vi "Test_HelloWorld_InvalidUtf8Encoding.vi"() -> (0 "Array of Error Description":T1)   [LabVIEW 2019]
uses:
  gRPC_ATS/TestUtility/utility.llb/array of error description.ctl
  gRPC_ATS/TestUtility/utility.llb/error description.ctl
  gRPC_ATS/TestUtility/utility.llb/error type.ctl
  examples/helloworld/helloworld_client/RPC Messages/helloworld_HelloRequest.ctl
  690210b7-9fc1-4805-899f-f09b8e1640af.vi
  86c0777a-bec3-4a03-9553-2f9525a5fa02.vi
  <vilib>/gRPC/LabVIEW gRPC Library/Server API/Translate Protobuf Error.vi
  <vilib>/AdvancedString/1D String Array to Delimited String.vi
  <vilib>/gRPC/LabVIEW gRPC Library/Server API/Server/Get Server DLL Path.vi
  examples/helloworld/helloworld_client/helloworld_client.lvlib
panel:
  out "Pass":bool
  in  "error in (no error)":errorcluster
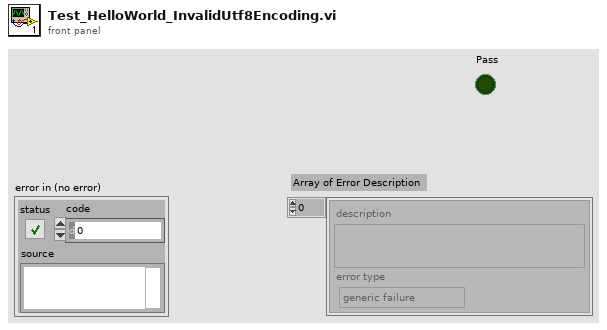
[diagram p1: front panel]
types:
  T1 = typedef "array of error description.ctl" = T2[]
  T2 = typedef "error description.ctl" = cluster{"description":string, "error type":T3}
  T3 = typedef "error type.ctl" = enum32{"generic failure", "boundary case", "precision", "expected error"}
  T4 = typedef "helloworld_client.lvlib/helloworld_HelloRequest.ctl" = cluster{"name":string}
  T5 = typedef "grpc-lvsupport-release.lvlib/grpcId.ctl" = u64
  T6 = typedef "grpc-lvsupport-release.lvlib/Any.ctl" = cluster{"Type Url":string, "Bytes":u8[]}
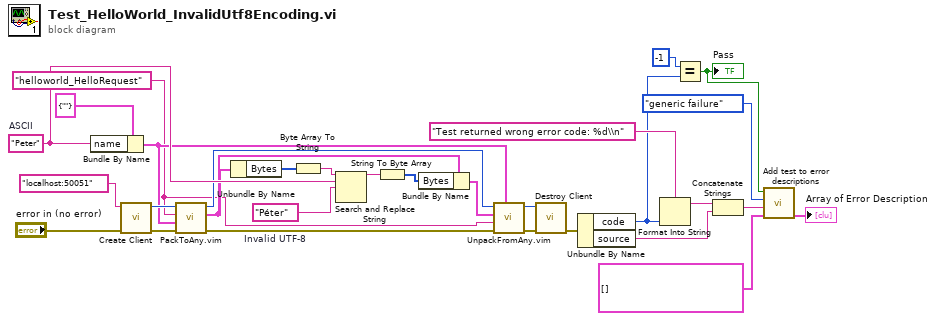
[diagram p0: block diagram]
diagram:
  w16 = "Péter"  # Invalid UTF-8
  w17 = "Peter"  # ASCII
  w9 = "helloworld_HelloRequest" ("Message Type")
  n1 = Bundle By Name(cluster=T4 {"name"=""} ("helloworld_HelloRequest"), "name"=w17) -> (w11:T4)
  n2 = call "Create Client.vi"("error in"="error in (no error)", "address"="localhost:50051") -> ("error out"=w23:errorcluster, "gRPC ID Out"=w22:T5)  [unwired: 8 in]
  n3 = call "PackToAny.vim"("error in"=w23, "Data To Pack"=w11, "Message Type"=w9, "gRPCid in"=w22) -> ("error out"=w7:errorcluster, "Any"=w14:T6, "gRPCid out"=w10:u64)  [unwired: 5 in]
  n4 = Unbundle By Name(w14) -> ("Bytes"=w19:u8[])
  n5 = Byte Array To String(unsigned byte array=w19) -> (string=w18:string)
  n6 = Search and Replace String(input string=w18, search string=w17, replace string=w16) -> (result string=w15:string)  [unwired: 5 in, 3 out]
  n7 = String To Byte Array(string=w15) -> (unsigned byte array=w13:u8[])
  n8 = Bundle By Name(cluster=w14, "Bytes"=w13) -> (w12:T6)
  n9 = call "UnpackFromAny.vim"("Data Type"=w11, "error in"=w7, "Message Type"=w9, "Any"=w12, "gRPCid in"=w10) -> ("error out"=w5:errorcluster, "gRPCid out"=w8:u64)  [unwired: 4 in, 1 out]
  n10 = call "Destroy Client.vi"("error in"=w5, "gRPC ID"=w8) -> ("error out"=w6:errorcluster)  [unwired: 9 in]
  n11 = Unbundle By Name(w6) -> ("code"=w2:i32, "source"=w25:string)
  n12 = Format Into String(format string="Test returned wrong error code: %d\\n" ("string"), w2) -> (resulting string=w1:string)  [unwired: 2 in, 1 out]
  n13 = Equal?(x=-1, y=w2) -> (x = y?=w27:bool)
  "Pass" <- w27
  n14 = Concatenate Strings(w1, w25) -> (w26:string)
  n15 = call "Add test to error descriptions.vi"("error descriptions in"=T1 [], "error string"=w26, "error type"=error_type."generic failure", "pass"=w27) -> ("error description out"=→"Array of Error Description":T1)  [unwired: 3 in]
